vi "niSwitch Detach gRPC Session.vi"(8 "error in":errorcluster, 11 "session factory in":refnum<class "Session Factory.lvclass">) -> (0 "error out":errorcluster)   [LabVIEW 2021, in "Session Management niSwitch.lvlib" / "Session Factory.lvclass"]
doc: "Detaches from the gRPC session specified in <b>session factory in</b>."
uses:
  Session Factory.lvclass
  Session Factory.lvclass/Session Factory.ctl
  NI Switch Client/NI Switch Client.lvlib
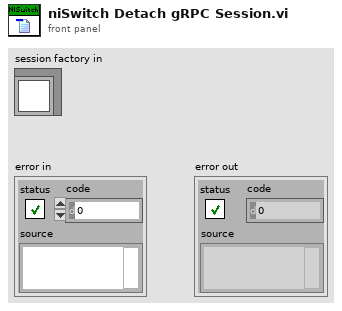
[diagram p1: front panel]
types:
  T1 = typedef "grpc-lvsupport-release.lvlib/grpcId.ctl" = u64
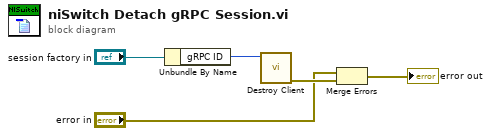
[diagram p0: block diagram]
diagram:
  n1 = Unbundle By Name("session factory in") -> ("gRPC ID"=w5:T1)
  n2 = call "Destroy Client.vi"("gRPC ID"=w5) -> ("error out"=w4:errorcluster)  [unwired: 10 in]
  n3 = Merge Errors("error in", w4) -> (→"error out":errorcluster)
